vi "FuncVI-DialogBoxSL.vi"(5 "InstanceRef":T2, 9 "arg list":T1[](array[typedef]) {"num" format="%.2f"}) -> (0 "error out":bool, 3 "result":T1 {"num" format="%.2f"})   [LabVIEW 2021]
doc: "::: CalcExpress Toolkit :::\nCopyright (c) 2000-2026 Konstantin Shifershteyn. All rights reserved."
uses:
  cetypes.llb/CalcExpress Function Argument Info.ctl
  cetypes.llb/CalcExpress Instance RefNum.ctl
panel:
  in  "max arg num":i32=1000
  in  "min arg num":i32=1
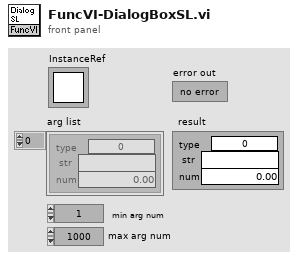
[diagram p1: front panel]
types:
  T1 = typedef "CalcExpress Function Argument Info.ctl" = cluster{"type":u32, "str":string, "num":dbl}
  T2 = typedef "CalcExpress Instance RefNum.ctl" = refnum<k1>
  T3 = enum8{"String", "DBL Number", "identifier", "1D Array of DBL", "2D Array of DBL", "CDB Number", "1D Array of CDB", "2D Array of CDB", "Unknown data type"}
  T4 = typedef "VarMan Variable Context Handle.ctl" = i32
  T5 = cluster{"var type":enum8{"String", "DBL Number", "identifier", "1D Array of DBL", "2D Array of DBL", "CDB Number", "1D Array of CDB", "2D Array of CDB", "Unknown data type"}, string, dbl}
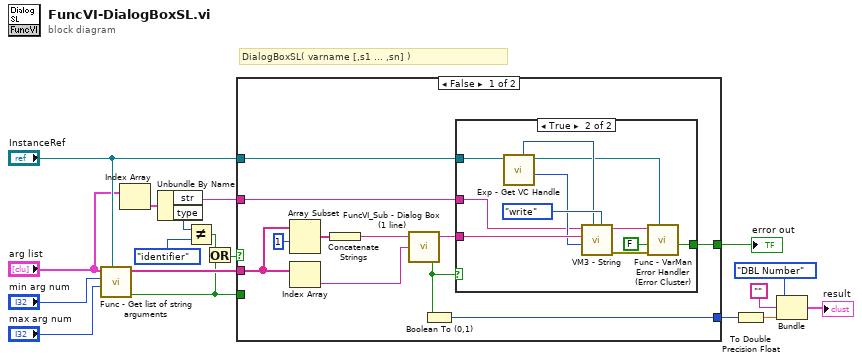
[diagram p0: block diagram]
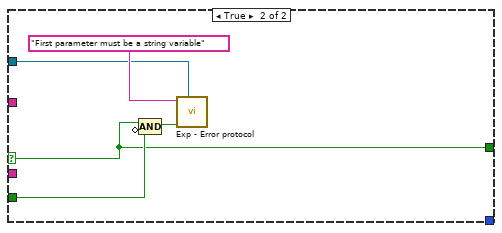
[diagram p3: hidden frame]
diagram:
  # "DialogBoxSL( varname [,s1 ... ,sn] )"
  n1 = call "Func - Get list of string arguments.vi"("InstanceRef"="InstanceRef", "max arg num"="max arg num", "min arg num"="min arg num", "arg list"="arg list") -> ("error out"=w10:bool, "val list"=w18:string[])  [unwired: 4 in]
  n2 = Index Array(array="arg list") -> (element=w11:T1)  [unwired: 1 in]
  n3 = Unbundle By Name(w11) -> ("str"=w3:string, "type"=w12:u32)
  n4 = Not Equal?(x=w12, y=T3."identifier" ("var type")) -> (x != y?=w13:bool)
  n5 = Or(x=w13, y=w10) -> (x .or. y?=w15:bool)
  n6 = case shown="False" w15 {
    selector: w15 -> [_ w44]
    tunnel: w18 -> [w26 _]
    tunnel: [w28 _] -> w7
    tunnel: "InstanceRef" -> [w23 w41]
    tunnel: [w21 w44] -> w16
    tunnel: w3 -> [w22 _]
    tunnel: w10 -> [_ w45]
    frame False {
      n7 = Array Subset(array=w26, index=1) -> (w25:string[])  [unwired: 1 in]
      n8 = Index Array(array=w26) -> (element=w27:string)  [unwired: 1 in]
      n9 = Concatenate Strings(w25) -> (w24:string)
      n10 = call "FuncVI_Sub - Dialog Box (1 line).vi"("data"=w27, "message"=w24) -> ("True ?"=w19:bool, "string out"=w20:string)  [unwired: 2 in]
      n11 = Boolean To (0,1)(Boolean=w19) -> (0, 1=w28:i16)
      n12 = case shown="True" w19 {
        tunnel: w23 -> [_ w40]
        tunnel: [_ w33] -> w21
        tunnel: w20 -> [_ w35]
        tunnel: w22 -> [_ w30]
        frame False {
        }
        frame True {
          n13 = call "Exp - Get VC Handle.vi"("InstanceRef"=w40) -> ("writer ID"=w34:u32, "dup InstanceRef"=w31:T2, "VC Handle"=w36:T4)  [unwired: 5 in, 1 out]
          n14 = call "VM3 - String.vi"("cmd (read)"=enum16{"create", "destroy", "write", "read"}."write", "VC Handle"=w36, "writer ID"=w34, "value in"=w35, "name_spec"=w30) -> ("error out"=w39:errorcluster, "dup name_spec"=w38:string)  [unwired: 3 in, 2 out]
          n15 = call "Func - VarMan Error Handler (Error Cluster).vi"("InstanceRef"=w31, "VarMan VI error in"=w39, "error status before"=FALSE, "var name"=w38) -> ("FuncVI error out"=w33:bool)  [unwired: 5 in, 2 out]
        }
      }
    }
    frame True {
      n16 = Compound Arithmetic op=AND(w44, invert w45) -> (w43:bool)
      n17 = call "Exp - Error protocol.vi"("InstanceRef"=w41, "error in"=w43, "error message in"="First parameter must be a string variable") -> ()  [unwired: 5 in, 2 out]
    }
  }
  "error out" <- w16
  n18 = To Double Precision Float(number=w7) -> (double precision float=w6:dbl)
  n19 = Bundle("var type"=T3."DBL Number", "", w6) -> (→"result":T5)  [unwired: 1 in]
